vi "Set Data Value.vi"(8 "error in (no error)":errorcluster, 9 "Flat Data":u8[](array[numeric]) format="%.0x", 11 "CIFTag in":refnum<class "CIF_Iceoryx_Chn_String.lvclass">) -> (0 "error out":errorcluster, 1 "Updated":bool, 3 "CIFTag out":refnum<class "CIF_Iceoryx_Chn_String.lvclass">)   [LabVIEW 2021, in "CIF_Iceoryx_Chn_String.lvclass"]
uses:
  CIF_Iceoryx_Chn_String.lvclass
  CIF_Iceoryx_Chn_String.lvclass/CIF_Iceoryx_Chn_String.ctl
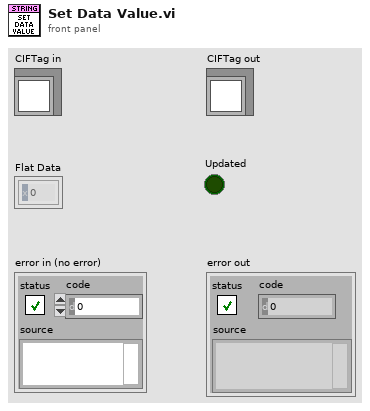
[diagram p1: front panel]
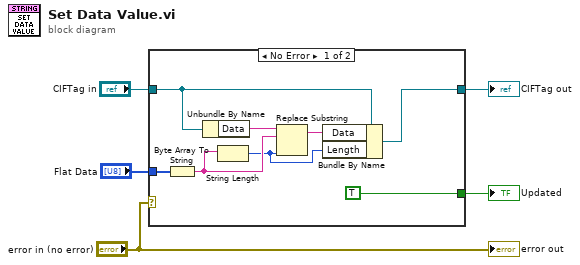
[diagram p0: block diagram]
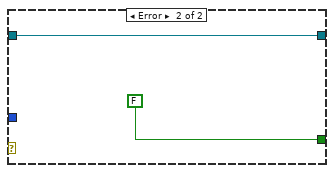
[diagram p2: hidden frame]
diagram:
  n1 = case shown="No Error" "error in (no error)" {
    tunnel: "Flat Data" -> [w11 _]
    tunnel: "CIFTag in" -> [w10 w15]
    tunnel: [w13 w15] -> w3
    tunnel: [TRUE FALSE] -> w2
    frame No Error {
      n2 = Byte Array To String(unsigned byte array=w11) -> (string=w8:string)
      n3 = Unbundle By Name(w10) -> ("Data"=w9:string)
      n4 = String Length(string=w8) -> (length=w6:i32)
      n5 = Replace Substring(2:w6, 4:w8, 5:w9) -> (1:w7:string)  [unwired: 1 in, 1 out]
      n6 = Bundle By Name(cluster=w10, "Data"=w7, "Length"=w6) -> (w13:refnum<class "CIF_Iceoryx_Chn_String.lvclass">)
    }
    frame Error {
    }
  }
  "CIFTag out" <- w3
  "Updated" <- w2
  "error out" <- "error in (no error)"
